vi "W18_Flash.vi"() -> ()   [LabVIEW 2018]
doc: "Use this template to build a VI to use as a subVI."
panel:
  out "error out":errorcluster
  out "flash OK":bool
  out "return code":i32
  out "output text":string
  in  "fw":string
  in  "tool":string
  # "tool: full path of STM32_Programmer_CLI.exe (or the fake: run W18_fake\\make_fake.cmd, then paste the path it prints)."
  # "fw names for the fake: ...nolink..., ...verifyfail..., ...masked... ; anything else = OK."
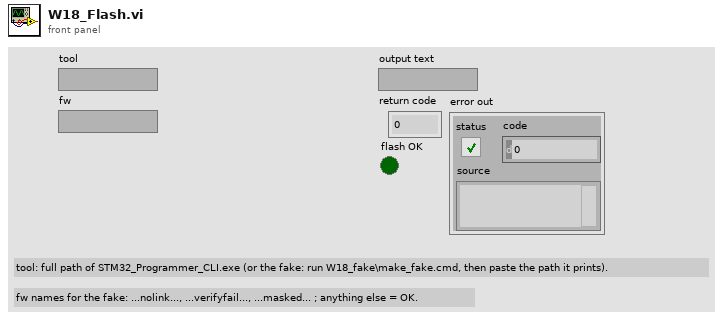
[diagram p1: front panel]
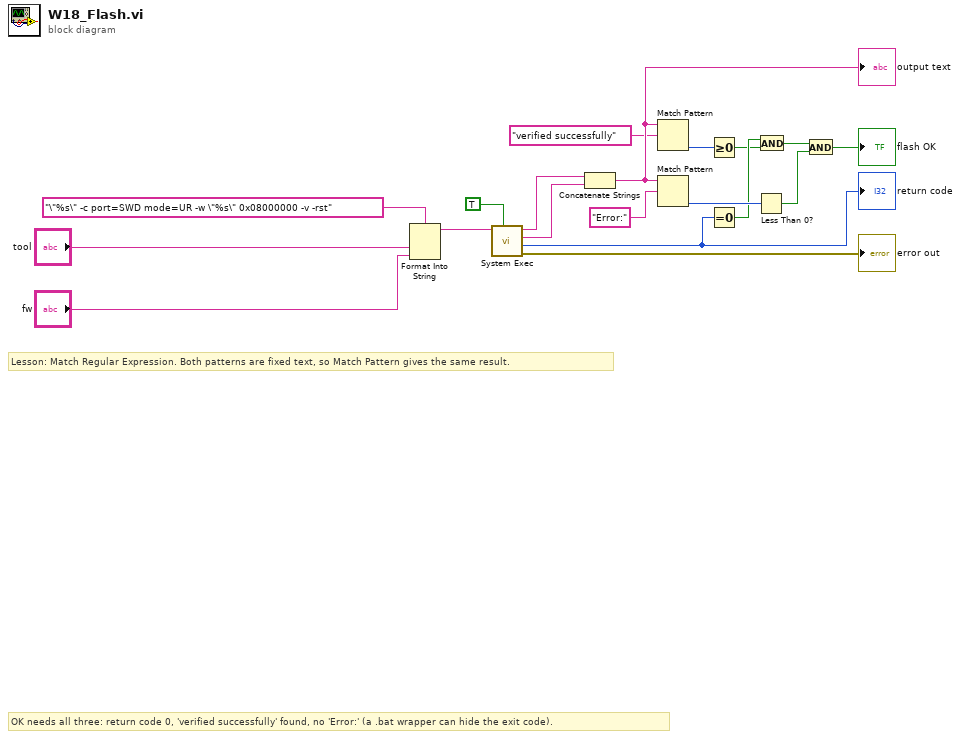
[diagram p0: block diagram]
diagram:
  # "OK needs all three: return code 0, 'verified successfully' found, no 'Error:' (a .bat wrapper can hide the exit code)."
  # "Lesson: Match Regular Expression. Both patterns are fixed text, so Match Pattern gives the same result."
  n1 = Format Into String(format string="\"%s\" -c port=SWD mode=UR -w \"%s\" 0x08000000 -v -rst", "tool", "fw") -> (resulting string=w16:string)  [unwired: 2 in, 1 out]
  n2 = call <vilib>:"System Exec.vi"("wait until completion? (T)"=TRUE, "command line"=w16) -> ("error out"=→"error out":errorcluster, "return code"=w7:i32, "standard error"=w13:string, "standard output"=w14:string)  [unwired: 6 in]
  "return code" <- w7
  n3 = Concatenate Strings(w14, w13) -> (w12:string)
  "output text" <- w12
  n4 = Match Pattern(string=w12, regular expression="verified successfully") -> (offset past match=w10:i32)  [unwired: 1 in, 3 out]
  n5 = Match Pattern(string=w12, regular expression="Error:") -> (offset past match=w8:i32)  [unwired: 1 in, 3 out]
  n6 = Greater Or Equal To 0?(x=w10) -> (x >= 0?=w5:bool)
  n7 = Equal To 0?(x=w7) -> (x = 0?=w6:bool)
  n8 = Less Than 0?(x=w8) -> (x < 0?=w3:bool)
  n9 = And(x=w6, y=w5) -> (x .and. y?=w4:bool)
  n10 = And(x=w4, y=w3) -> (x .and. y?=→"flash OK":bool)
